vi "CE Center.vi"(4 "var cmd":T4(ring)=enum."get value", 6 "exec":T5(ring)=enum."CalcExpress", 7 "VC Handle":T3=-1, 8 "error in":errorcluster, 10 "values in":T2={"type"=enum."DBL Number", "dbl"=0.0, "cdb"=0.0+0.0i, "str"="", "1d dbl"=[], "1d cdb"=[], "1d str"=[], "2d dbl"=[], "2d cdb"=[], "2d str"=[]} {"2d cdb" format="%.2f"; "2d dbl" format="%.2f"; "1d cdb" format="%.2f"; "1d dbl" format="%.2f"; "cdb" format="%.2f"; "dbl" format="%.2f"}, 11 "expression/name":string) -> (0 "error out":errorcluster, 2 "values out":T2={"type"=enum."DBL Number", "dbl"=0.0, "cdb"=0.0+0.0i, "str"="", "1d dbl"=[], "1d cdb"=[], "1d str"=[], "2d dbl"=[], "2d cdb"=[], "2d str"=[]} {"2d cdb" format="%.2f"; "2d dbl" format="%.2f"; "1d cdb" format="%.2f"; "1d dbl" format="%.2f"; "cdb" format="%.2f"; "dbl" format="%.2f"}, 5 "VC Handle out":T3=-1)   [LabVIEW 2021]
doc: "::: CalcExpress Toolkit :::\nCopyright (c) 2000-2026 Konstantin Shifershteyn. All rights reserved."
uses:
  vi.lib/addons/CalcExpress/cetypes.llb/VarMan Variable Context Handle.ctl
  vi.lib/addons/CalcExpress/cetypes.llb/CalcExpress Data Type.ctl
  vi.lib/addons/CalcExpress/cetypes.llb/VarMan Error Code.ctl
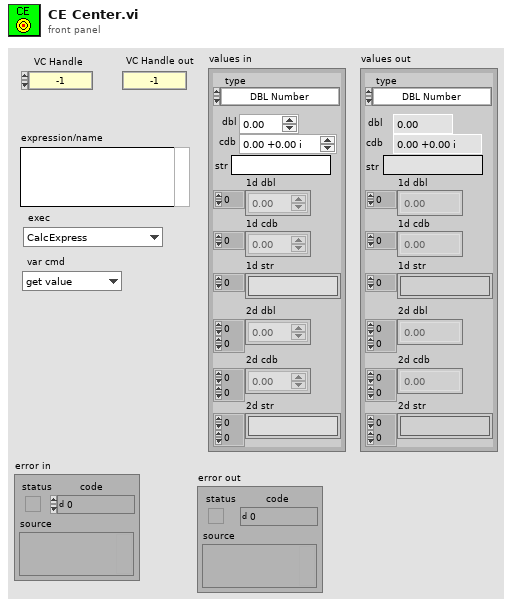
[diagram p1: front panel]
types:
  T1 = typedef "CalcExpress Data Type.ctl" = enum32{"String", "DBL Number", "identifier", "1D Array of DBL", "2D Array of DBL", "CDB Number", "1D Array of CDB", "2D Array of CDB", "1D Array of String", "2D Array of String", "Unknown data type"}
  T2 = cluster{"type":T1, "dbl":dbl, "cdb":cdb, "str":string, "1d dbl":dbl[], "1d cdb":cdb[], "1d str":string[], "2d dbl":dbl[][], "2d cdb":cdb[][], "2d str":string[][]}
  T3 = typedef "VarMan Variable Context Handle.ctl" = i32
  T4 = enum16{"create", "destroy", "set value", "get value"}
  T5 = enum16{"open session", "close session", "CalcExpress", "VarMan", "VarMan (low level)"}
  T6 = typedef "VarMan Error Code.ctl" = u16
  T7 = cluster{"type":enum32{"String", "DBL Number", "identifier", "1D Array of DBL", "2D Array of DBL", "CDB Number", "1D Array of CDB", "2D Array of CDB", "1D Array of String", "2D Array of String", "Unknown data type"}, "dbl":dbl, "cdb":cdb, "str":string, "1d dbl":dbl[], "1d cdb":cdb[], "1d str":string[], "2d dbl":dbl[][], "2d cdb":cdb[][], "2d str":string[][]}
  T8 = enum16{"ok", "invalid type", "var not def", "var already def", "inv handle", "input error", "invalid data format", "unknown error"}
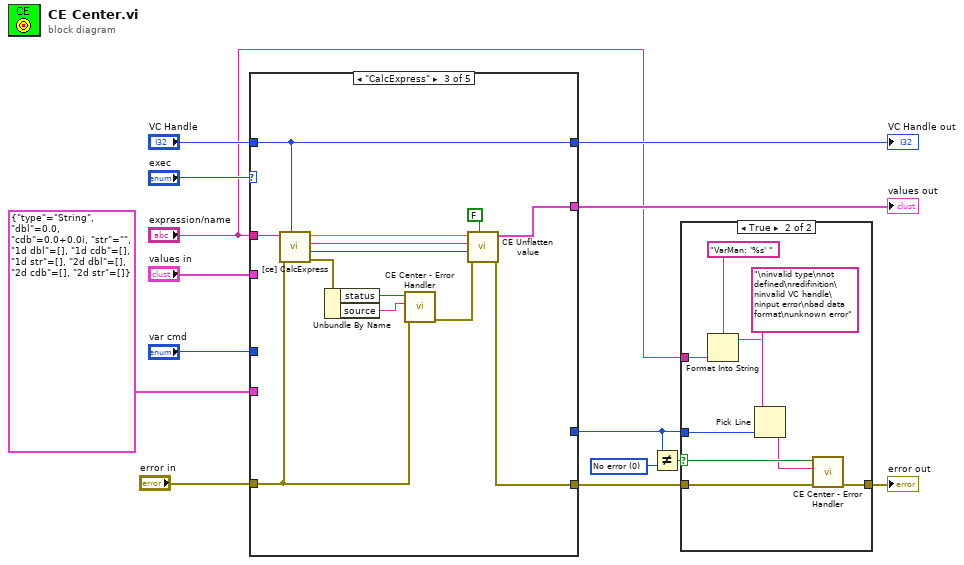
[diagram p0: block diagram]
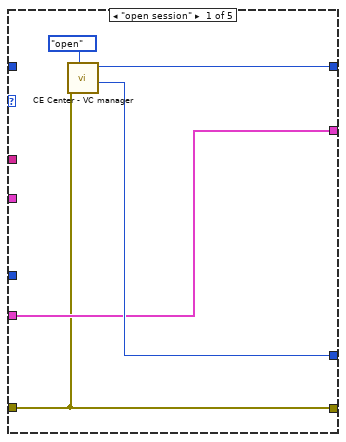
[diagram p3: hidden frame]
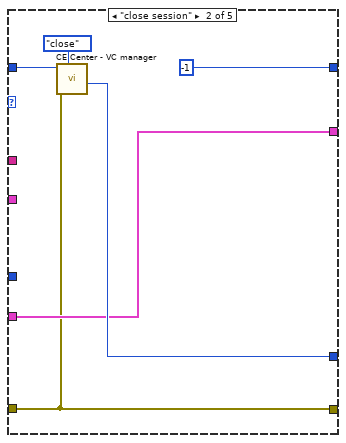
[diagram p4: hidden frame]
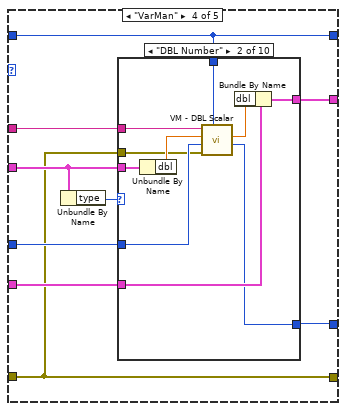
[diagram p5: hidden frame]
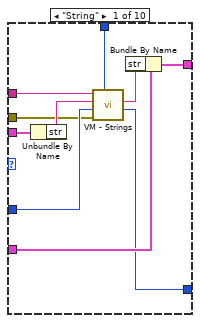
[diagram p6: hidden frame]
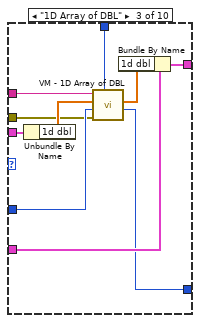
[diagram p7: hidden frame]
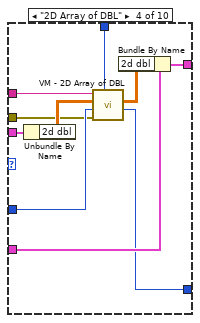
[diagram p8: hidden frame]
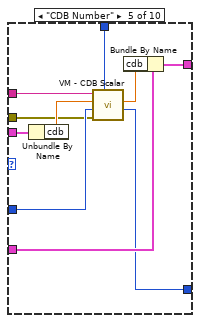
[diagram p9: hidden frame]
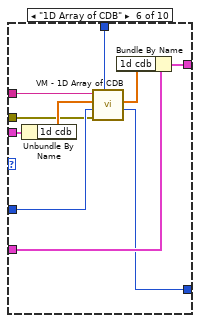
[diagram p10: hidden frame]
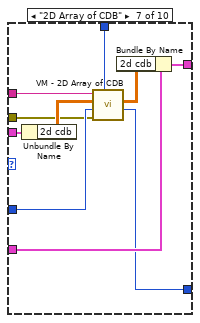
[diagram p11: hidden frame]
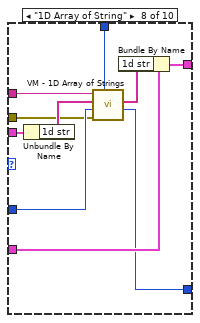
[diagram p12: hidden frame]
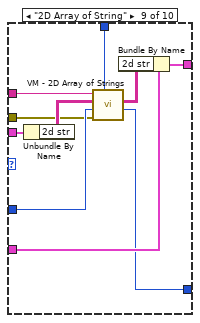
[diagram p13: hidden frame]
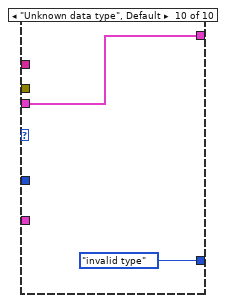
[diagram p14: hidden frame]
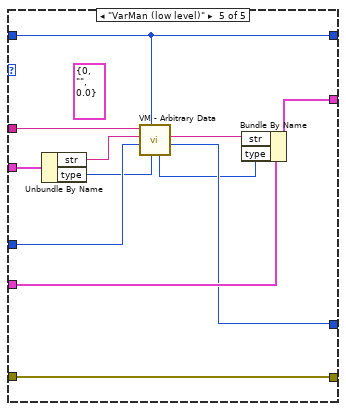
[diagram p15: hidden frame]
diagram:
  w2 = T6 0 items=["No error", "Invalid variable type", "Variable not found", "Variable already exists", "Invalid context handle", "Input error", "Invalid data format", "No history attached", "History already attached", "Invalid history parameters", "Wrong variable name", "Wrong alias name", "Non-unique alias", "Alias not found", "No alias associated", "Alias already associated", "Wrong context name", "Non-unique context name", "Context name not found", "Invalid parameter", "Generic error", "Memory Full", "Unrecognized LV error", "Unknown error code"] ("x")
  n1 = case shown="\"CalcExpress\"" "exec" {
    tunnel: "VC Handle" -> [_ w24 w38 w47 w143]
    tunnel: [w18 -1 ("VC Handle") w38 w47 w143] -> w12
    tunnel: [w15 w20 w32 w39 w148] -> w4
    tunnel: "expression/name" -> [_ _ w37 w42 w147]
    tunnel: T7 {"type"=enum."String", "dbl"=0.0, "cdb"=0.0+0.0i, "str"="", "1d dbl"=[], "1d cdb"=[], "1d str"=[], "2d dbl"=[], "2d cdb"=[], "2d str"=[]} ("values in") -> [w16 w21 _ w45 w150]
    tunnel: [w16 w21 w31 w46 w151] -> w11
    tunnel: "values in" -> [_ _ _ w44 w149]
    tunnel: [w19 w23 _ w41 w142] -> w1
    tunnel: "var cmd" -> [_ _ _ w40 w146]
    tunnel: "error in" -> [w15 w20 w29 w39 w148]
    frame "open session" {
      n2 = call "CE Center - VC manager.vi"("cmd"=enum16{"open", "close", "close all"}."open", "error in"=w15) -> ("err code"=w19:T6, "VC Handle out"=w18:T3)  [unwired: 5 in, 1 out]
    }
    frame "close session" {
      n3 = call "CE Center - VC manager.vi"("cmd"=enum16{"open", "close", "close all"}."close", "error in"=w20, "VC Handle"=w24) -> ("err code"=w23:T6)  [unwired: 4 in, 2 out]
    }
    frame "CalcExpress" {
      n4 = call "[ce] CalcExpress.vi"("VC Handle"=w38, "error in"=w29, "expression"=w37) -> ("error out"=w28:errorcluster, "value type"=w34:T1, "string value"=w35:string, "numeric value"=w36:dbl)  [unwired: 3 in]
      n5 = Unbundle By Name(w28) -> ("status"=w27:bool, "source"=w26:string)
      n6 = call "CE Center - Error Handler.vi"("error before"=w29, "CE message"=w26, "CE error status"=w27) -> ("error out"=w33:errorcluster)  [unwired: 6 in]
      n7 = call "CE Unflatten value.vi"("Flattened DBL?"=FALSE, "error in"=w33, "type"=w34, "flattened data"=w35, "dbl"=w36) -> ("error out"=w32:errorcluster, "values out"=w31:T2)  [unwired: 3 in]
    }
    frame "VarMan" {
      n8 = Unbundle By Name(w44) -> ("type"=w43:T1)
      n9 = case shown="\"DBL Number\"" w43 {
        tunnel: w47 -> [w57 w67 w77 w87 w97 w107 w117 w127 w137 _]
        tunnel: w42 -> [w56 w66 w76 w86 w96 w106 w116 w126 w136 _]
        tunnel: w39 -> [w48 w58 w68 w78 w88 w98 w108 w118 w128 _]
        tunnel: [w54 w64 w74 w84 w94 w104 w114 w124 w134 w139] -> w46
        tunnel: w45 -> [w52 w62 w72 w82 w92 w102 w112 w122 w132 _]
        tunnel: [w51 w61 w71 w81 w91 w101 w111 w121 w131 T8."invalid type" ("err code")] -> w41
        tunnel: w40 -> [w50 w60 w70 w80 w90 w100 w110 w120 w130 _]
        tunnel: w44 -> [w49 w59 w69 w79 w89 w99 w109 w119 w129 w139]
        frame "String" {
          n10 = Unbundle By Name(w49) -> ("str"=w55:string)
          n11 = call "VM - Strings.vi"("VC Handle"=w57, "error in"=w48, "cmd"=w50, "value in"=w55, "name_spec"=w56) -> ("err code"=w51:T6, "value out"=w53:string)  [unwired: 1 in, 4 out]
          n12 = Bundle By Name(cluster=w52, "str"=w53) -> (w54:T7)
        }
        frame "DBL Number" {
          n13 = Unbundle By Name(w59) -> ("dbl"=w65:dbl)
          n14 = call "VM - DBL Scalar.vi"("VC Handle"=w67, "error in"=w58, "cmd"=w60, "value in"=w65, "name_spec"=w66) -> ("err code"=w61:T6, "value out"=w63:dbl)  [unwired: 1 in, 4 out]
          n15 = Bundle By Name(cluster=w62, "dbl"=w63) -> (w64:T7)
        }
        frame "1D Array of DBL" {
          n16 = Unbundle By Name(w69) -> ("1d dbl"=w75:dbl[])
          n17 = call "VM - 1D Array of DBL.vi"("VC Handle"=w77, "error in"=w68, "cmd"=w70, "value in"=w75, "name_spec"=w76) -> ("err code"=w71:T6, "value out"=w73:dbl[])  [unwired: 1 in, 4 out]
          n18 = Bundle By Name(cluster=w72, "1d dbl"=w73) -> (w74:T7)
        }
        frame "2D Array of DBL" {
          n19 = Unbundle By Name(w79) -> ("2d dbl"=w85:dbl[][])
          n20 = call "VM - 2D Array of DBL.vi"("VC Handle"=w87, "error in"=w78, "cmd"=w80, "value in"=w85, "name_spec"=w86) -> ("err code"=w81:T6, "value out"=w83:dbl[][])  [unwired: 1 in, 4 out]
          n21 = Bundle By Name(cluster=w82, "2d dbl"=w83) -> (w84:T7)
        }
        frame "CDB Number" {
          n22 = Unbundle By Name(w89) -> ("cdb"=w95:cdb)
          n23 = call "VM - CDB Scalar.vi"("VC Handle"=w97, "error in"=w88, "cmd"=w90, "value in"=w95, "name_spec"=w96) -> ("err code"=w91:T6, "value out"=w93:cdb)  [unwired: 1 in, 4 out]
          n24 = Bundle By Name(cluster=w92, "cdb"=w93) -> (w94:T7)
        }
        frame "1D Array of CDB" {
          n25 = Unbundle By Name(w99) -> ("1d cdb"=w105:cdb[])
          n26 = call "VM - 1D Array of CDB.vi"("VC Handle"=w107, "error in"=w98, "cmd"=w100, "value in"=w105, "name_spec"=w106) -> ("err code"=w101:T6, "value out"=w103:cdb[])  [unwired: 1 in, 4 out]
          n27 = Bundle By Name(cluster=w102, "1d cdb"=w103) -> (w104:T7)
        }
        frame "2D Array of CDB" {
          n28 = Unbundle By Name(w109) -> ("2d cdb"=w115:cdb[][])
          n29 = call "VM - 2D Array of CDB.vi"("VC Handle"=w117, "error in"=w108, "cmd"=w110, "value in"=w115, "name_spec"=w116) -> ("err code"=w111:T6, "value out"=w113:cdb[][])  [unwired: 1 in, 4 out]
          n30 = Bundle By Name(cluster=w112, "2d cdb"=w113) -> (w114:T7)
        }
        frame "1D Array of String" {
          n31 = Unbundle By Name(w119) -> ("1d str"=w125:string[])
          n32 = call "VM - 1D Array of Strings.vi"("VC Handle"=w127, "error in"=w118, "cmd"=w120, "value in"=w125, "name_spec"=w126) -> ("err code"=w121:T6, "value out"=w123:string[])  [unwired: 1 in, 4 out]
          n33 = Bundle By Name(cluster=w122, "1d str"=w123) -> (w124:T7)
        }
        frame "2D Array of String" {
          n34 = Unbundle By Name(w129) -> ("2d str"=w135:string[][])
          n35 = call "VM - 2D Array of Strings.vi"("VC Handle"=w137, "error in"=w128, "cmd"=w130, "value in"=w135, "name_spec"=w136) -> ("err code"=w131:T6, "value out"=w133:string[][])  [unwired: 1 in, 4 out]
          n36 = Bundle By Name(cluster=w132, "2d str"=w133) -> (w134:T7)
        }
        frame "Unknown data type", Default {
        }
      }
    }
    frame "VarMan (low level)" {
      (unwired) cluster{"type":u8, "str":string, "num":dbl} {"type"=0, "str"="", "num"=0.0} ("par in")
      n37 = Unbundle By Name(w149) -> ("str"=w145:string, "type"=w144:T1)
      n38 = call "VM - Arbitrary Data.vi"("var type"=w144, "VC Handle"=w143, "cmd"=w146, "flattened value"=w145, "name_spec"=w147) -> ("err code"=w142:T6, "flattened value out"=w141:string, "var type out"=w140:u32)  [unwired: 1 in, 3 out]
      n39 = Bundle By Name(cluster=w150, "str"=w141, "type"=w140) -> (w151:T7)
    }
  }
  "VC Handle out" <- w12
  "values out" <- w11
  n40 = Not Equal?(x=w1, y=w2) -> (x != y?=w8:bool)
  n41 = case shown="True" w8 {
    selector: w8 -> [_ w154]
    tunnel: w1 -> [_ w160]
    tunnel: "expression/name" -> [_ w157]
    tunnel: w4 -> [w152 w156]
    tunnel: [w152 w155] -> w3
    frame False {
    }
    frame True {
      n42 = Format Into String(format string="VarMan: '%s' " ("string (\"\")"), w157) -> (resulting string=w158:string)  [unwired: 2 in, 1 out]
      n43 = Pick Line(string ("")=w158, multi-line string="\ninvalid type\nnot defined\nredifinition\ninvalid VC handle\ninput error\nbad data format\nunknown error", line index=w160) -> (output string=w153:string)
      n44 = call "CE Center - Error Handler.vi"("error before"=w156, "CE message"=w153, "CE error status"=w154) -> ("error out"=w155:errorcluster)  [unwired: 6 in]
    }
  }
  "error out" <- w3
